vi "Start Periodic Enqueue Message.vi"(6 "Period [ms]":i32, 8 "error in (no error)":errorcluster, 9 "Message Data":variant, 10 "Message":string, 11 "MHL Queue":refnum<class "Delacor_lib_QMH_Message Queue.lvclass">) -> (0 "error out":errorcluster, 3 "Helper Loop":refnum<class "Helper Loop DQMH.lvclass">)   [LabVIEW 2026, in "Helper Loop DQMH.lvclass"]
doc: "入力したメッセージキュー、メッセージ、データ、周期で周期処理を開始します。\n無限待機中のヘルパーループが存在する場合はそのうちの1つを使用し、なければユーザーイベントを作成してヘルパーループを呼び出します。"
uses:
  Helper Loop DQMH.lvclass
  Helper Loop DQMH.lvclass/Helper Loop DQMH.ctl
  OneDrive/HP/Local/DQMH Helper/Helper Loop/Sub/Helper Loop Core.vi
  OneDrive/HP/Local/DQMH Helper/Helper Loop/Sub/Helper Loop Map FGV Action.ctl
  <vilib>/Delacor/Delacor QMH/Libraries/Message Queue_class/Delacor_lib_QMH_Message Queue.lvclass
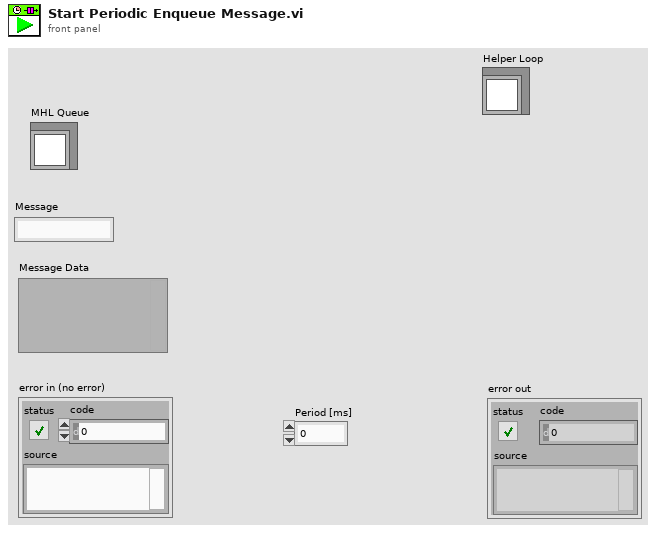
[diagram p1: front panel]
types:
  T1 = typedef "Helper Loop DQMH.lvclass/Helper Loop Map FGV Action.ctl" = enum16{"Get Pausing Helper Loop", "Register Active Helper Loop", "Pause Helper Loop", "Close Helper Loop", "Get All Helper Loops"}
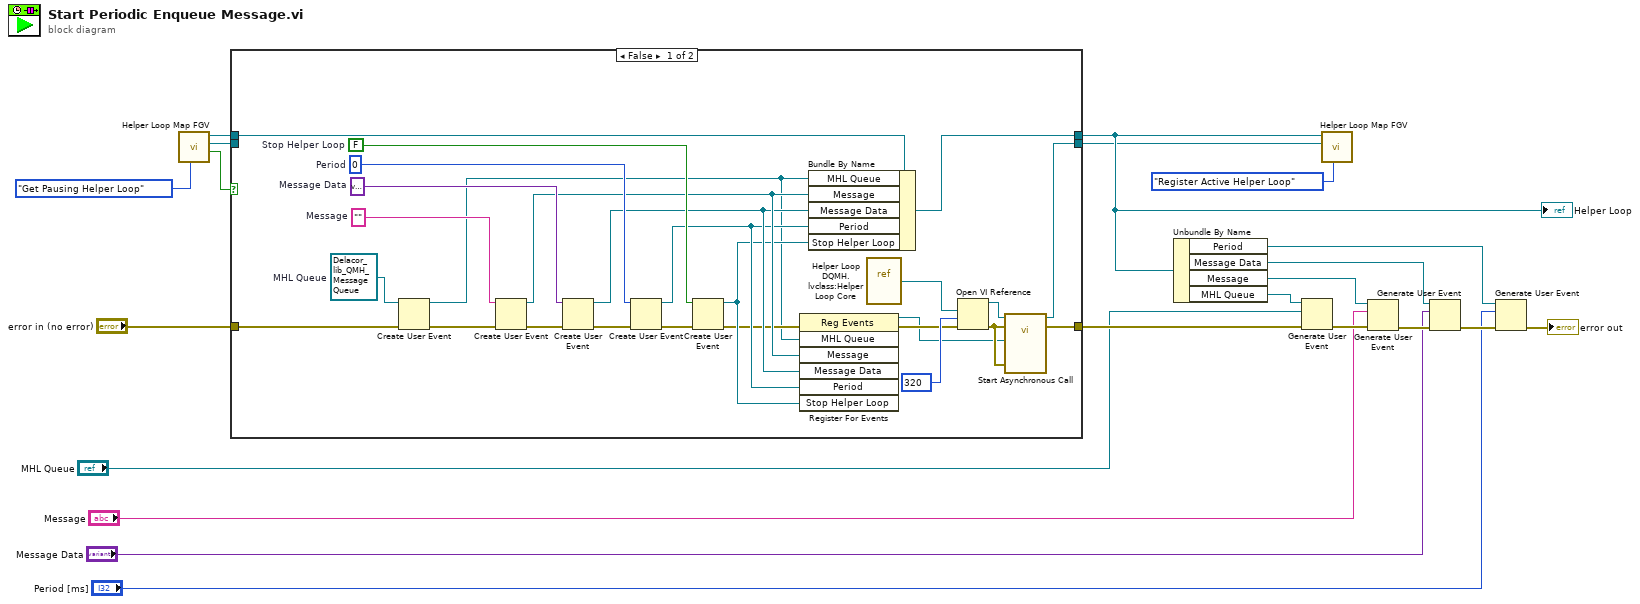
[diagram p0: block diagram]
diagram:
  n1 = call "Helper Loop Map FGV.vi"("Action"=Helper_Loop_Map_FGV_Action."Get Pausing Helper Loop") -> ("Get Helper Loop"=w8:bool, "Helper Loop VI Reference Out"=w4:refnum<vi>, "Helper Loop Out"=w7:refnum<class "Helper Loop DQMH.lvclass">)  [unwired: 7 in, 1 out]
  n2 = case shown="False" w8 {
    tunnel: "error in (no error)" -> [w35 w49]
    tunnel: [w34 w49] -> w2
    tunnel: [w32 w50] -> w5
    tunnel: w7 -> [w33 w50]
    tunnel: w4 -> [_ w48]
    tunnel: [w22 w48] -> w3
    frame False {
      w24 = refnum<class "Delacor_lib_QMH_Message Queue.lvclass"> refnum  # MHL Queue
      w38 = FALSE  # Stop Helper Loop
      w43 = 0  # Period
      w44 = variant  # Message Data
      w45 = ""  # Message
      n3 = Create User Event(user event datatype=w24, error in=w35) -> (user event=w25:refnum<user-event>, error out=w42:errorcluster)
      n4 = Create User Event(user event datatype=w45, error in=w42) -> (user event=w31:refnum<user-event>, error out=w41:errorcluster)
      n5 = Create User Event(user event datatype=w44, error in=w41) -> (user event=w30:refnum<user-event>, error out=w40:errorcluster)
      n6 = Create User Event(user event datatype=w43, error in=w40) -> (user event=w29:refnum<user-event>, error out=w39:errorcluster)
      n7 = Create User Event(user event datatype=w38, error in=w39) -> (user event=w28:refnum<user-event>, error out=w27:errorcluster)
      n8 = register-events(error in=w27, w25, w31, w30, w29, w28) -> (reference out=w23:refnum<event-registration>, error out=w26:errorcluster)  [unwired: 1 in]
      n9 = Bundle By Name(cluster=w33, "MHL Queue"=w25, "Message"=w31, "Message Data"=w30, "Period"=w29, "Stop Helper Loop"=w28) -> (w32:refnum<class "Helper Loop DQMH.lvclass">)
      n10 = vi-ref "Helper Loop DQMH.lvclass:Helper Loop Core.vi"() -> (w46:refnum<vi>)
      n11 = Open VI Reference(vi path=w46, options=320, error in (no error)=w26) -> (vi reference=w37:refnum<vi>, error out=w36:errorcluster)  [unwired: 3 in]
      n12 = call-by-ref "Start Asynchronous Call"(reference=w37, error in=w36, "error in"=w36, "Event Registration Refnum"=w23) -> (reference out=w22:refnum<vi>, error out=w34:errorcluster)  [unwired: 9 in, 1 out]
    }
    frame True {
    }
  }
  "Helper Loop" <- w5
  n13 = Unbundle By Name(w5) -> ("Period"=w17:refnum<user-event>, "Message Data"=w16:refnum<user-event>, "Message"=w15:refnum<user-event>, "MHL Queue"=w14:refnum<user-event>)
  n14 = Generate User Event(user event=w14, event data cluster="MHL Queue", error in=w2) -> (error out=w20:errorcluster)  [unwired: 1 in, 1 out]
  n15 = call "Helper Loop Map FGV.vi"("Action"=Helper_Loop_Map_FGV_Action."Register Active Helper Loop", "Helper Loop VI Reference In"=w3, "Helper Loop In"=w5) -> ()  [unwired: 5 in, 4 out]
  n16 = Generate User Event(user event=w15, event data cluster="Message", error in=w20) -> (error out=w18:errorcluster)  [unwired: 1 in, 1 out]
  n17 = Generate User Event(user event=w16, event data cluster="Message Data", error in=w18) -> (error out=w19:errorcluster)  [unwired: 1 in, 1 out]
  n18 = Generate User Event(user event=w17, event data cluster="Period [ms]", error in=w19) -> (error out=→"error out":errorcluster)  [unwired: 1 in, 1 out]
